vi "FMV - set cluster element.vi"(8 "error in (no error)":errorcluster, 11 "JSON string":string) -> (0 "error out":errorcluster, 3 "value":string)   [LabVIEW 2020, in "ui-testing.lvlib"]
doc: "copyright: Thomas Zilliox©"
uses:
  ui-testing.lvlib
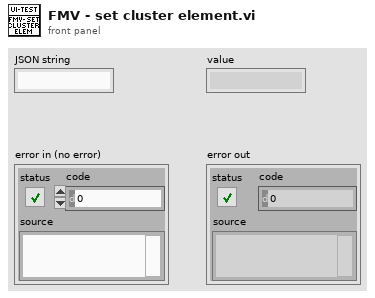
[diagram p1: front panel]
types:
  T1 = cluster{"name":string, "type":string, "value":string, "layers":string[]}
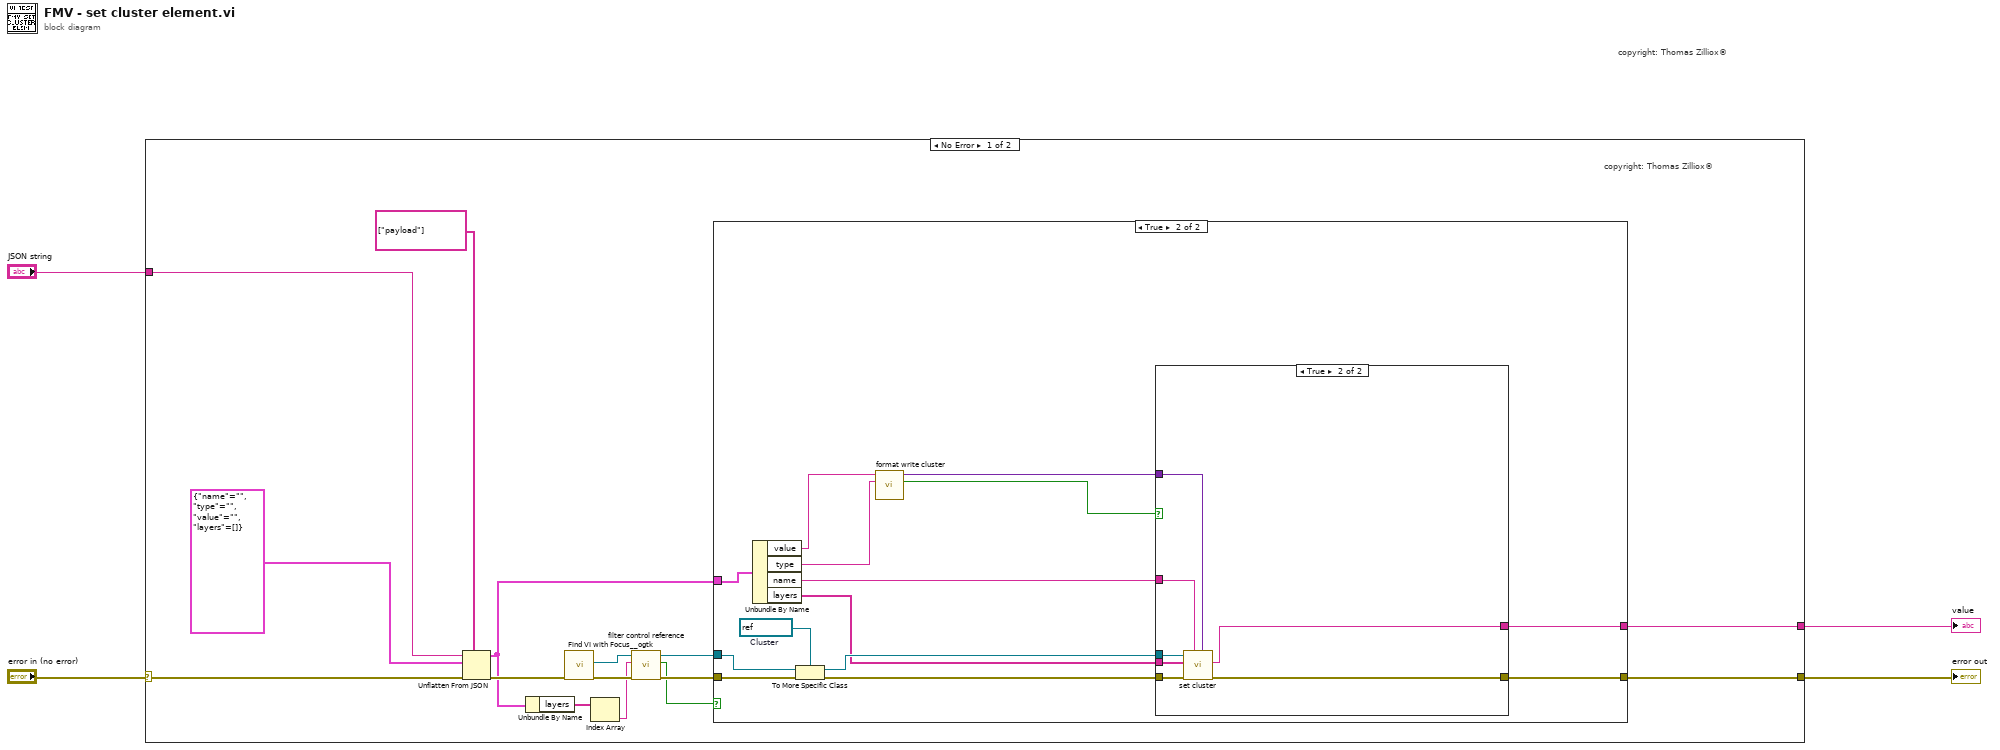
[diagram p0: block diagram]
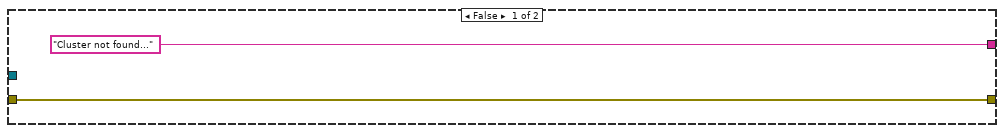
[diagram p2: hidden frame]
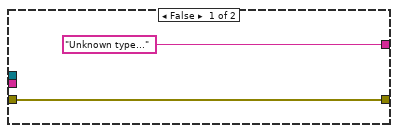
[diagram p3: hidden frame]
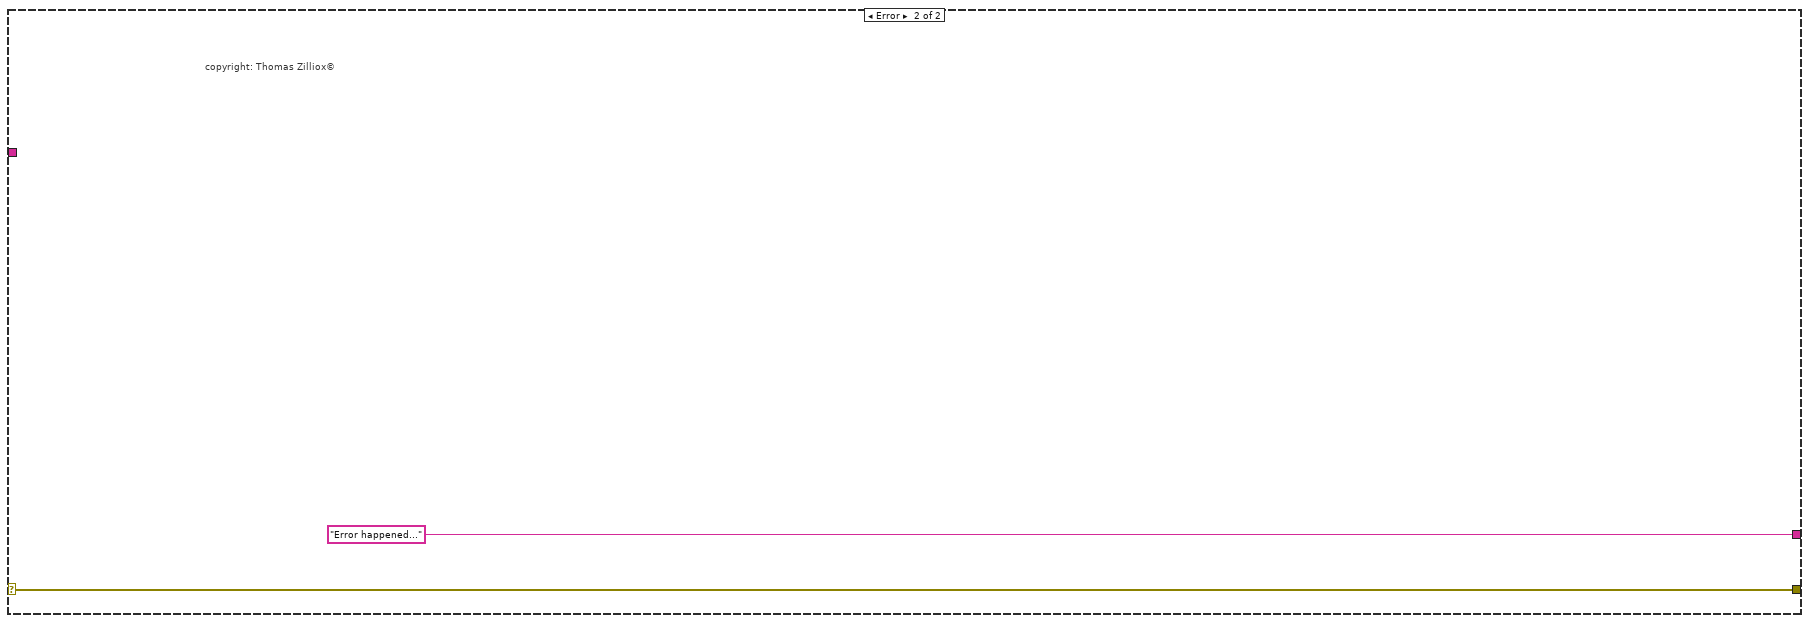
[diagram p4: hidden frame]
diagram:
  # "copyright: Thomas Zilliox©"
  n1 = case shown="No Error" "error in (no error)" {
    selector: "error in (no error)" -> [w17 w46]
    tunnel: "JSON string" -> [w18 _]
    tunnel: [w6 w46] -> w3
    tunnel: [w7 "Error happened..."] -> w2
    frame No Error {
      # "copyright: Thomas Zilliox©"
      n2 = Unflatten From JSON(path=string[] ["payload"], JSON string=w18, type and defaults=T1 {"name"="", "type"="", "value"="", "layers"=[]}, error in (no error)=w17) -> (value=w5:T1, error out=w16:errorcluster)  [unwired: 3 in]
      n3 = Unbundle By Name(w5) -> ("layers"=w12:string[])
      n4 = call <userlib>:"Find VI with Focus__ogtk.vi"("error in"=w16) -> ("error out"=w14:errorcluster, "VI with Focus"=w13:refnum<vi>)  [unwired: 6 in, 3 out]
      n5 = Index Array(array=w12) -> (element=w11:string)  [unwired: 1 in]
      n6 = call "filter control reference.vi"("error in (no error)"=w14, "Control label"=w11, "VI (Caller)"=w13) -> ("error out"=w9:errorcluster, "Control found"=w8:bool, "Control ref"=w10:refnum<vi>)  [unwired: 6 in]
      n7 = case shown="True" w8 {
        tunnel: w10 -> [_ w32]
        tunnel: w9 -> [w21 w35]
        tunnel: [w21 w34] -> w6
        tunnel: ["Cluster not found..." w26] -> w7
        tunnel: w5 -> [_ w29]
        frame False {
        }
        frame True {
          w30 = refnum<vi> refnum  # Cluster
          n8 = Unbundle By Name(w29) -> ("value"=w25:string, "type"=w24:string, "name"=w27:string, "layers"=w28:string[])
          n9 = To More Specific Class(target class=w30, reference=w32, error in=w35) -> (specific class reference=w31:refnum<vi>, error out=w33:errorcluster)
          n10 = call "format write cluster.vi"("type"=w24, "value"=w25) -> ("Valid ?"=w22:bool, "Variant"=w23:variant)  [unwired: 8 in]
          n11 = case shown="True" w22 {
            tunnel: [w37 w44] -> w34
            tunnel: w33 -> [w37 w43]
            tunnel: w31 -> [_ w42]
            tunnel: w28 -> [_ w41]
            tunnel: w27 -> [_ w40]
            tunnel: ["Unknown type..." w38] -> w26
            tunnel: w23 -> [_ w39]
            frame False {
            }
            frame True {
              n12 = call "set cluster.vi"("Value"=w39, "Label"=w40, "error in (no error)"=w43, "Layer arrary"=w41, "cluster ref"=w42) -> ("error out"=w44:errorcluster, "Acknowledge message"=w38:string)  [unwired: 5 in]
            }
          }
        }
      }
    }
    frame Error {
      # "copyright: Thomas Zilliox©"
    }
  }
  "error out" <- w3
  "value" <- w2
